vi "Test Overflow.vi"(8 "error in":errorcluster, 11 "Test Case In":refnum<class "History Tests.lvclass">) -> (0 "error out":errorcluster, 3 "Test Case Out":refnum<class "History Tests.lvclass">)   [LabVIEW 2020, in "History Tests.lvclass"]
doc: "Adds many states to the undo buffer and then performs an Undo on all of the added states."
uses:
  History Tests.lvclass
  History Tests.lvclass/History Tests.ctl
  <vilib>/Astemes/LUnit/Test Case.lvclass
  resource/plugins/NIIconEditor/History/History/History.lvclass
panel:
  out "Have Changes":bool
  out "Undo Data":string[](array[string])
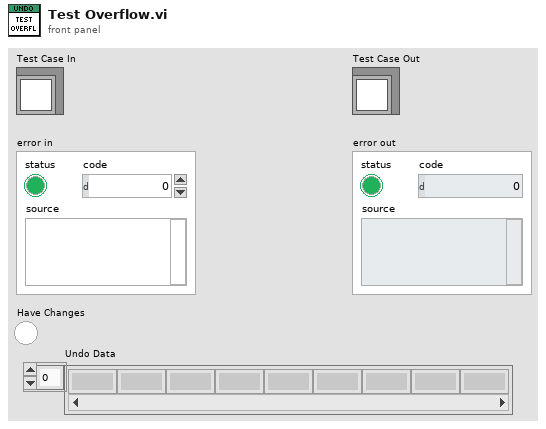
[diagram p1: front panel]
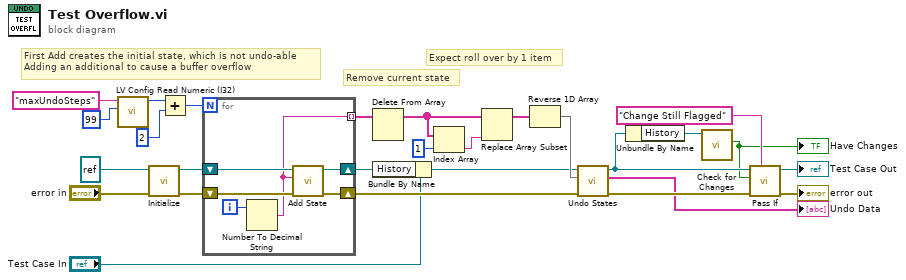
[diagram p0: block diagram]
diagram:
  # "Expect roll over by 1 item"
  # "Remove current state"
  # "First Add creates the initial state, which is not undo-able\nAdding an additional to cause a buffer overflow"
  n1 = call <resource>:"LV Config Read Numeric (I32).vi"("default value"=99, "key"="maxUndoSteps") -> ("value"=w19:i32)  [unwired: 3 in, 2 out]
  n2 = call "Initialize.vi"("error in"="error in", "menu reference"=refnum<k9> refnum) -> ("error out"=w24:errorcluster, "History"=w7:refnum<class "History.lvclass">)  [unwired: 8 in]
  n3 = Add(x=w19, y=2) -> (x+y=w18:i32)
  n4 = for {
    N: w18 -> [_]
    tunnel: [w28] -> w16 mode=indexing
    shift-right: [w29] -> w6
    shift-left: w7 -> [w30]
    shift-right: [w32] -> w23
    shift-left: w24 -> [w33]
    i -> [w31]
    n5 = Number To Decimal String(number=w31) -> (decimal integer string=w28:string)  [unwired: 1 in]
    n6 = call "Add State.vi"("error in"=w33, "State"=w28, "History in"=w30) -> ("error out"=w32:errorcluster, "History out"=w29:refnum<class "History.lvclass">)  [unwired: 7 in]
  }
  n7 = Delete From Array(array=w16) -> (array with subset deleted=w9:string[])  [unwired: 2 in, 1 out]
  n8 = Bundle By Name(cluster="Test Case In", "History"=w6) -> (w4:refnum<class "History Tests.lvclass">)
  n9 = Index Array(array=w9, index=1) -> (element=w14:string)
  n10 = Replace Array Subset(array=w9, new element=w14) -> (w13:string[])  [unwired: 1 in]
  n11 = Reverse 1D Array(array=w13) -> (reversed array=w10:string[])
  n12 = call "Undo States.vi"("error in"=w23, "Expected Undo States"=w10, "Test Case In"=w4) -> ("error out"=w27:errorcluster, "Actual Undo States"=→"Undo Data":string[], "Test Case Out"=w3:refnum<class "History Tests.lvclass">)  [unwired: 6 in]
  n13 = Unbundle By Name(w3) -> ("History"=w2:refnum<class "History.lvclass">)
  n14 = call "Check for Changes.vi"("History"=w2) -> ("Have Changes"=w1:bool)  [unwired: 10 in]
  "Have Changes" <- w1
  n15 = call <vilib>:"Pass If.vi"("Description"="Change Still Flagged", "error in (no error)"=w27, "Pass?"=w1, "LUnit Test Case In"=w3) -> ("error out"=→"error out":errorcluster, "LUnit Test Case Out"=→"Test Case Out":refnum<class "History Tests.lvclass">)  [unwired: 6 in]
